vi "Map Extension Examples.vi"() -> ()   [LabVIEW 2020]
uses:
  6012eb03-068b-47dd-84b2-e47ab68c7cda.vi
  d52ac117-3a0c-4c38-a035-cd1ec790ca6a.vi
  158e93f0-6d83-44df-a97f-fd033c23c3c4.vi
  9f2e02d3-5876-4709-beaf-12703edb0216.vi
  0236d640-7fb0-4049-b526-a4a0acec0d8d.vi
  77e0272d-242f-412b-982f-1600aba21800.vi
  8d18f84e-651b-4bc2-8d26-9827fa866315.vi
  332644c8-09cd-45c9-9348-425bf23ac390.vi
  14195457-9666-4654-9939-676a4b3105cd.vi
  6012eb03-068b-47dd-84b2-e47ab68c7cda.vi/68c40cae-4346-4630-a6b2-e0fb86e48665.vi
  9f2e02d3-5876-4709-beaf-12703edb0216.vi/b0178052-0c48-4c9a-874f-40b592e34ac5.vi
  77e0272d-242f-412b-982f-1600aba21800.vi/8ee94aa7-4836-4e87-a0a7-557d81cff62b.vi
panel:
  out "Converted (Associated) Arrays to Map?":bool
  out "key found?":bool
  out "Created Empty Map?":bool
  out "keys":string[](array[string])
  out "Keys":i32[](array[numeric])
  out "Converted Array to Map?":bool
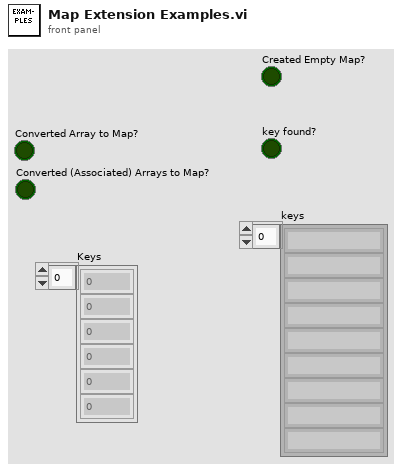
[diagram p1: front panel]
types:
  T1 = cluster{"bool":bool, "string":string, "bool 2":bool, "Name":i32}
  T2 = map{string, cluster{"bool":bool, "string":string, "bool 2":bool, "Name":i32}}
  T3 = cluster{i32[], cluster{"bool":bool, "string":string}[]}
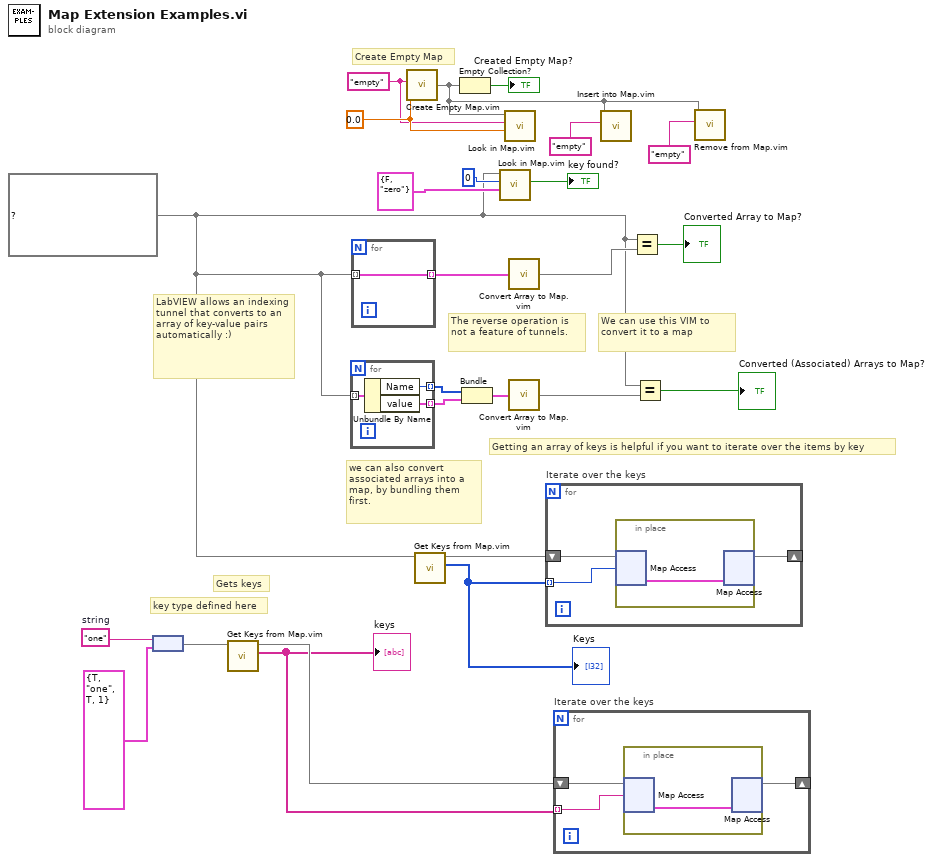
[diagram p0: block diagram]
diagram:
  w3 = map{i32, cluster{"bool":bool, "string":string}} {0={"bool"=FALSE, "string"="zero"}, 1={"bool"=TRUE, "string"="one"}} ("map out")
  w13 = 0.0
  w10 = "empty" ("key type")
  w19 = "one"  # string
  # "we can also convert associated arrays into a map, by bundling them first."
  # "Getting an array of keys is helpful if you want to iterate over the items by key"
  # "key type defined here"
  # "Gets keys"
  # "We can use this VIM to convert it to a map"
  # "The reverse operation is not a feature of tunnels."
  # "Create Empty Map"
  # "LabVIEW allows an indexing tunnel that converts to an array of key-value pairs automatically :)"
  n1 = node(w19, T1 {"bool"=TRUE, "string"="one", "bool 2"=TRUE, "Name"=1}) -> (w18:T2)
  n2 = call "Get Keys from Map.vim"("map"=w18) -> ("keys"=w15:string[], "map out"=w16:T2)  [unwired: 9 in]
  "keys" <- w15
  n3 = for {
    tunnel: w3 -> [w28] mode=indexing
    tunnel: [w27] -> w6 mode=indexing
    tunnel: [w26] -> w5 mode=indexing
    n4 = Unbundle By Name(w28) -> ("Name"=w27:i32, "value"=w26:cluster{"bool":bool, "string":string})
  }
  n5 = for {
    tunnel: [w29] -> w25 mode=indexing
    tunnel: w3 -> [w29] mode=indexing
  }
  n6 = call "Create Empty Map.vim"("value type"=w13, "key type"=w10) -> ("empty map"=w8:map{string, dbl})  [unwired: 8 in]
  n7 = call "Get Keys from Map.vim"("map"=w3) -> ("keys"=w22:i32[], "map out"=w21:map{i32, cluster{"bool":bool, "string":string}})  [unwired: 9 in]
  "Keys" <- w22
  n8 = Empty Collection?(1:w8) -> (0:→"Created Empty Map?":bool)
  n9 = Bundle(w6, w5) -> (w4:T3)  [unwired: 1 in]
  n10 = call "Look in Map.vim"("default value"=cluster{"bool":bool, "string":string} {"bool"=FALSE, "string"="zero"} ("value"), "key"=0 ("Name"), "map"=w3) -> ("key found?"=→"key found?":bool)  [unwired: 7 in, 1 out]
  n11 = call "Look in Map.vim"("default value"=w13, "key"=w10, "map"=w8) -> ()  [unwired: 7 in, 2 out]
  n12 = call "Convert Array to Map.vim"("array"=w25) -> ("map"=w24:map{i32, cluster{"bool":bool, "string":string}})  [unwired: 6 in]
  n13 = call "Convert Array to Map.vim"("array"=w4) -> ("map"=w2:map{i32, cluster{"bool":bool, "string":string}})  [unwired: 6 in]
  n14 = for "Iterate over the keys" {
    shift-right: [w30] -> _
    shift-left: w21 -> [w31]
    tunnel: w22 -> [w32] mode=indexing
    n15 = in-place {
      n16 = in-place-map #1(w31, w32) -> (w33:cluster{"bool":bool, "string":string})  [unwired: 1 in, 1 out]
      n17 = in-place-map #1(w33) -> (w30:map{i32, cluster{"bool":bool, "string":string}})  [unwired: 1 in, 2 out]
    }
  }
  n18 = for "Iterate over the keys" {
    shift-right: [w34] -> _
    shift-left: w16 -> [w35]
    tunnel: w15 -> [w36] mode=indexing
    n19 = in-place {
      n20 = in-place-map #2(w35, w36) -> (w37:T1)  [unwired: 1 in, 1 out]
      n21 = in-place-map #2(w37) -> (w34:T2)  [unwired: 1 in, 2 out]
    }
  }
  n22 = call "Insert into Map.vim"("key"="empty" ("key type"), "map"=w8) -> ()  [unwired: 7 in, 3 out]
  n23 = Equal?(x=w3, y=w24) -> (x = y?=→"Converted Array to Map?":bool)
  n24 = Equal?(x=w3, y=w2) -> (x = y?=→"Converted (Associated) Arrays to Map?":bool)
  n25 = call "Remove from Map.vim"("key"="empty" ("key type"), "map"=w8) -> ()  [unwired: 7 in, 3 out]
